vi "query SCPI Command.vi"(8 "error in (no error)":errorcluster, 9 "Read Buffer Length":u32, 10 "SCPI Command":string, 11 "NR in":refnum<class "NR.lvclass">) -> (0 "error out":errorcluster, 2 "Read Buffer String":string, 3 "NR out":refnum<class "NR.lvclass">)   [LabVIEW 2023, in "ANRITSU Call Box.lvlib" / "NR.lvclass"]
uses:
  NR.lvclass
  NR.lvclass/NR.ctl
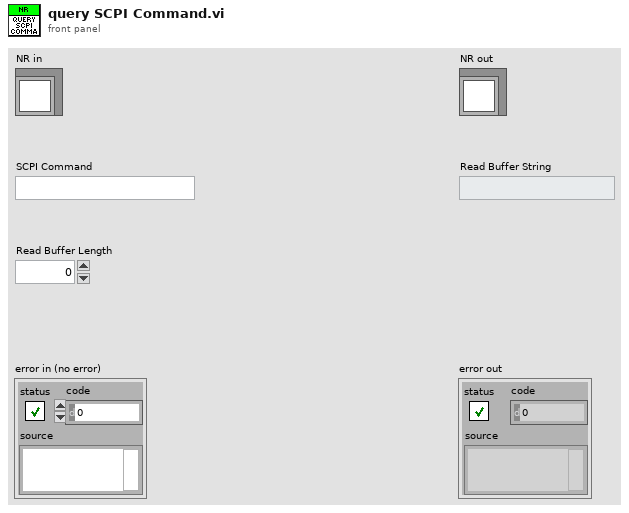
[diagram p1: front panel]
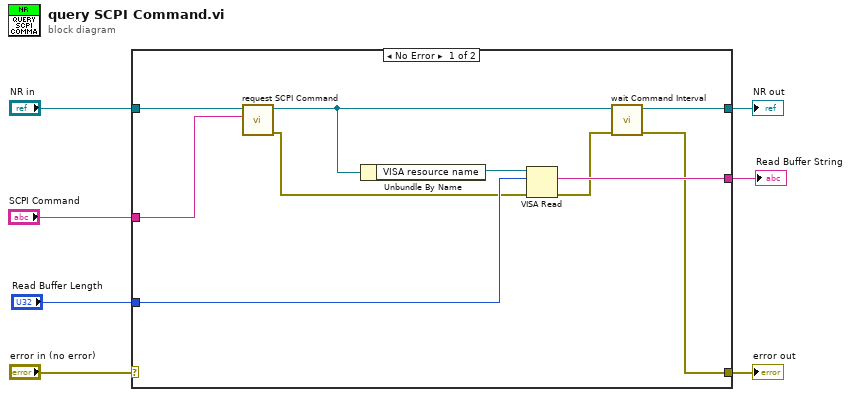
[diagram p0: block diagram]
diagram:
  n1 = case shown="No Error" "error in (no error)" {
    selector: "error in (no error)" -> [_ w19]
    tunnel: [w8 w19] -> w6
    tunnel: [w10 w18] -> w4
    tunnel: "NR in" -> [w17 w18]
    tunnel: "SCPI Command" -> [w16 _]
    tunnel: "Read Buffer Length" -> [w14 _]
    tunnel: [w12 _] -> w1
    frame No Error {
      n2 = call "request SCPI Command.vi"("SCPI Command"=w16, "NR in"=w17) -> ("error out"=w13:errorcluster, "NR out"=w11:refnum<class "NR.lvclass">)  [unwired: 8 in]
      n3 = Unbundle By Name(w11) -> ("VISA resource name"=w15:refnum<visa-resource-name>)
      n4 = VISA Read(VISA resource name=w15, byte count=w14, error in (no error)=w13) -> (read buffer=w12:string, error out=w9:errorcluster)  [unwired: 2 out]
      n5 = call "wait Command Interval.vi"("error in (no error)"=w9, "NR in"=w11) -> ("error out"=w8:errorcluster, "NR out"=w10:refnum<class "NR.lvclass">)  [unwired: 8 in]
    }
    frame Error {
    }
  }
  "error out" <- w6
  "NR out" <- w4
  "Read Buffer String" <- w1
